vi "Native_GetTerminalWire.vi"() -> ()   [LabVIEW 2024]
panel:
  out "error out":errorcluster caption="错误输出"
  out "wire_id":u32
  in  "wire_id type":u32
  in  "terminal_id":u32
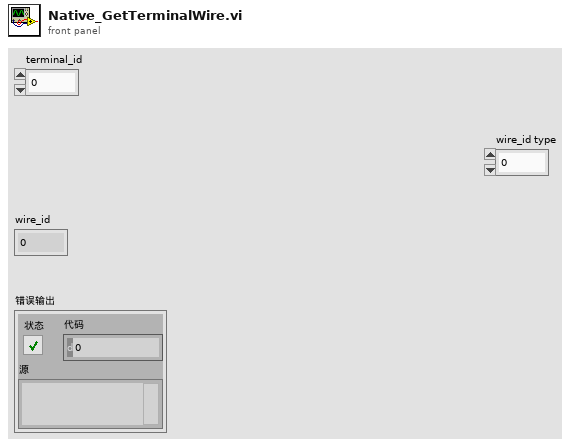
[diagram p1: front panel]
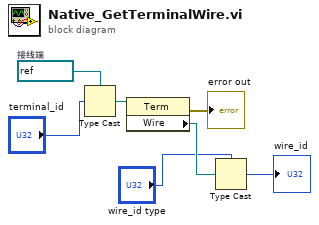
[diagram p0: block diagram]
diagram:
  w6 = refnum<vi> refnum  # 接线端
  n1 = Type Cast ("强制类型转换")(type=w6, x="terminal_id") -> (*(type *) &x=w5:refnum<vi>)
  n2 = property on="属性节点" class="Term"(reference=w5) -> (error out=→"error out":errorcluster, "Wire"=w4:refnum<vi>)  [unwired: 1 in, 1 out]
  n3 = Type Cast ("强制类型转换")(type="wire_id type", x=w4) -> (*(type *) &x=→"wire_id":u32)
